vi "Encode Frame.vi"(8 "error in":errorcluster, 10 "payload":string, 11 "packet_type":u8) -> (0 "error out":errorcluster, 3 "frame bytes":string)   [LabVIEW 2015, in "Lengmur_socket.lvlib"]
uses:
  Lengmur_socket.lvlib
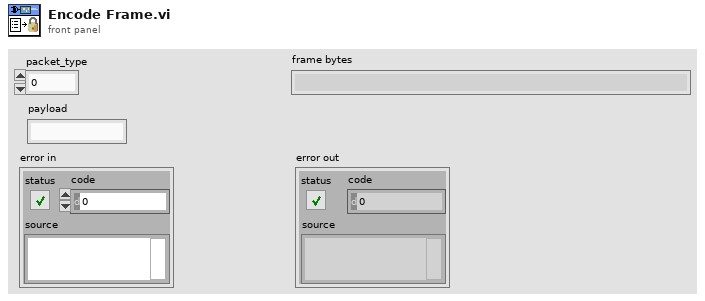
[diagram p1: front panel]
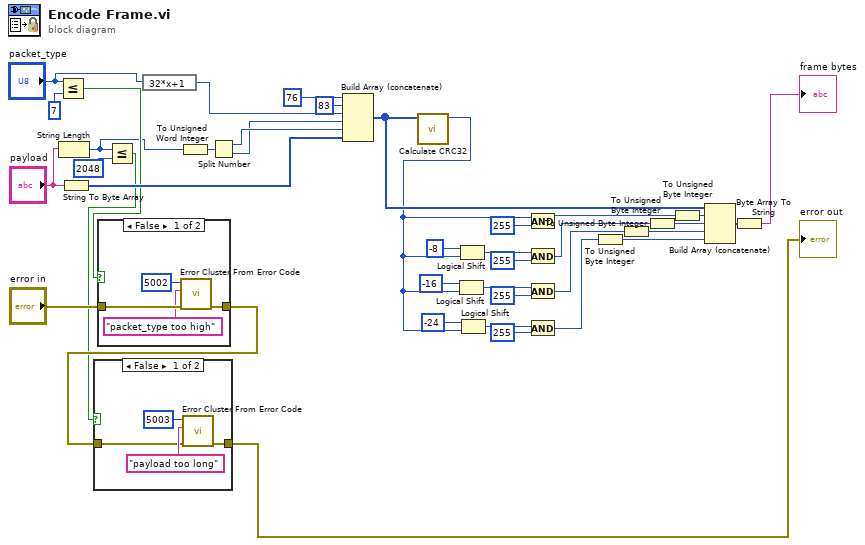
[diagram p0: block diagram]
diagram:
  n1 = Less Or Equal?(x="packet_type", y=u8 7) -> (x <= y?=w11:bool)
  n2 = String Length(string="payload") -> (length=w6:i32)
  n3 = String To Byte Array(string="payload") -> (unsigned byte array=w38:u8[])
  n4 = case shown="False" w11 {
    tunnel: [w43 w44] -> w8
    tunnel: "error in" -> [w42 w44]
    frame False {
      n5 = call <vilib>:"Error Cluster From Error Code.vi"("error in (no error)"=w42, "error message (\"\")"="packet_type too high" ("error message (\"\")"), "error code (0)"=5002) -> ("error out"=w43:errorcluster)  [unwired: 6 in]
    }
    frame True {
    }
  }
  n6 = Less Or Equal?(x=w6, y=2048) -> (x <= y?=w7:bool)
  n7 = case shown="False" w7 {
    tunnel: [w45 w49] -> w9
    tunnel: w8 -> [w46 w49]
    frame False {
      n8 = call <vilib>:"Error Cluster From Error Code.vi"("error in (no error)"=w46, "error message (\"\")"="payload too long" ("error message (\"\")"), "error code (0)"=5003) -> ("error out"=w45:errorcluster)  [unwired: 6 in]
    }
    frame True {
    }
  }
  "error out" <- w9
  n9 = expression code="32*x+1"("packet_type") -> (w35:u8)
  n10 = To Unsigned Word Integer(number=w6) -> (unsigned 16bit integer=w15:u16)
  n11 = Split Number(x=w15) -> (hi(x)=w17:u8, lo(x)=w16:u8)
  n12 = Build Array (concatenate)(u8 76 ("element"), u8 83 ("element"), w35, w16, w17, w38) -> (w2:u8[])
  n13 = call "Calculate CRC32.vi"("data bytes"=w2) -> ("crc32"=w1:u32)  [unwired: 9 in, 1 out]
  n14 = Logical Shift(y=-16 ("x"), x=w1) -> (x << y=w20:u32)
  n15 = Logical Shift(y=-8 ("x"), x=w1) -> (x << y=w22:u32)
  n16 = Logical Shift(y=-24 ("x"), x=w1) -> (x << y=w21:u32)
  n17 = And(x=w1, y=u32 255) -> (x .and. y?=w26:u32)
  n18 = And(x=w22, y=u32 255) -> (x .and. y?=w25:u32)
  n19 = And(x=w20, y=u32 255) -> (x .and. y?=w24:u32)
  n20 = And(x=w21, y=u32 255) -> (x .and. y?=w23:u32)
  n21 = To Unsigned Byte Integer(number=w23) -> (unsigned 8bit integer=w31:u8)
  n22 = To Unsigned Byte Integer(number=w24) -> (unsigned 8bit integer=w32:u8)
  n23 = To Unsigned Byte Integer(number=w25) -> (unsigned 8bit integer=w33:u8)
  n24 = To Unsigned Byte Integer(number=w26) -> (unsigned 8bit integer=w34:u8)
  n25 = Build Array (concatenate)(w2, w34, w33, w32, w31) -> (w19:u8[])
  n26 = Byte Array To String(unsigned byte array=w19) -> (string=→"frame bytes":string)
